vi "Stop Core.vi"(10 "final error code":i32, 11 "WebSocket Connection in":refnum<class "WebSocket Connection.lvclass">) -> (3 "WebSocket Connection out":refnum<class "WebSocket Connection.lvclass">)   [LabVIEW 2021, in "WebSocket Actors.lvlib" / "WebSocket Connection.lvclass"]
doc: "(<B>Filename</B>: Actor Framework.lvlib:Actor.lvclass:Stop Core.vi)\n\nDefines what the actor does before it stops. Use the <B>final error code</B> input to determine whether the actor shut down in response to an error.\n\nBy default, this method does nothing. A descendant class may override it to define behavior, such as shutting down any processes the actor initiated in its override of the Actor Core method."
uses:
  WebSocket Connection.lvclass
  Abstract Messages/WebSocket Connection Handler Msg/typedefs/Message Data.ctl
  <vilib>/ActorFramework/Message Enqueuer/Message Enqueuer.lvclass
  <vilib>/LS Instruments AG/LV-WebSockets/Data Format.ctl
  WebSocket Connection.lvclass/WebSocket Connection.ctl
  Abstract Messages/WebSocket Connection Handler Msg/properties/Connection Event.ctl
  <vilib>/LS Instruments AG/LV-WebSockets/StatusCode.ctl
  Abstract Messages/WebSocket Connection Handler Msg/WebSocket Connection Handler Msg.lvclass/WebSocket Connection Handler Msg.ctl
  <vilib>/ActorFramework/Message Enqueuer/Message Enqueuer.lvclass/Message Enqueuer.ctl
  <vilib>/ActorFramework/Message Enqueuer/Enqueue.vi
  Abstract Messages/WebSocket Connection Handler Msg/WebSocket Connection Handler Msg.lvclass
  C:/Program Files/National Instruments/LabVIEW 2021/vi.lib/ActorFramework/Message/Message.lvclass
  <vilib>/Utility/LVClass/Get LV Class Name.vi
  <resource>/AFDebug/Generate Trace for Message.vi
  <vilib>/ActorFramework/Message Priority Queue/Priority Enqueue.vi
  <vilib>/ActorFramework/Actor/Actor.lvclass
  <vilib>/LS Instruments AG/LV-WebSockets/LV WebSockets.lvlib
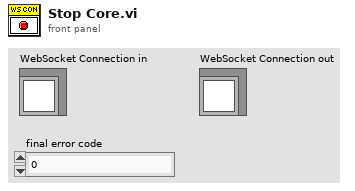
[diagram p1: front panel]
types:
  T1 = typedef "WebSocket Actors.lvlib/WebSocket Connection Handler Msg.lvclass/Message Data.ctl" = cluster{"Data":string, "Peer ID":string, "Connection Enqueuer":refnum<class "Message Enqueuer.lvclass">, "Data Format":T2}
  T2 = typedef "LV WebSockets.lvlib/Data Format.ctl" = enum16{"Text", "Binary"}
  T3 = typedef "WebSocket Actors.lvlib/WebSocket Connection.lvclass/Connection Status.ctl" = enum16{"Open", "Closed by Self", "Closed by Peer", "Dropped"}
  T4 = typedef "WebSocket Actors.lvlib/WebSocket Connection Handler Msg.lvclass/Connection Event.ctl" = enum16{"On Connect", "On Message", "On Close", "On Drop"}
  T5 = typedef "LV WebSockets.lvlib/StatusCode.ctl" = u16
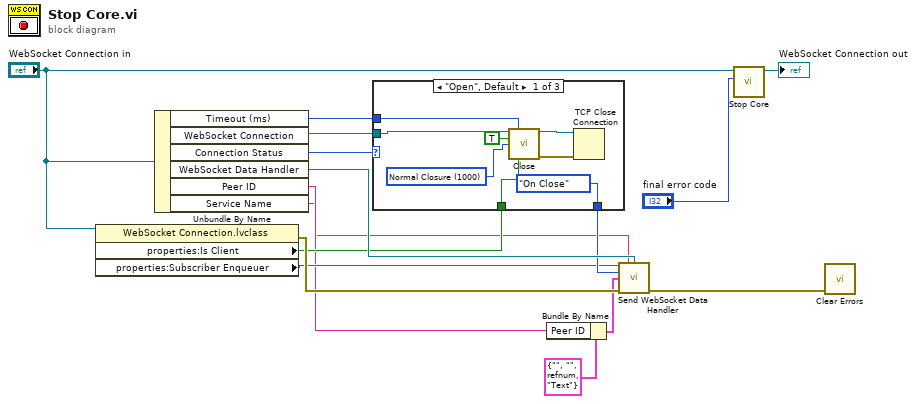
[diagram p0: block diagram]
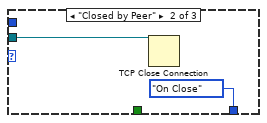
[diagram p2: hidden frame]
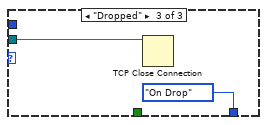
[diagram p3: hidden frame]
diagram:
  n1 = property class="WebSocket Connection.lvclass"(reference="WebSocket Connection in") -> (error out=w8:errorcluster, "properties:Is Client"=w6:bool, "properties:Subscriber Enqueuer"=w7:refnum<class "Message Enqueuer.lvclass">)  [unwired: 1 in, 1 out]
  n2 = Unbundle By Name("WebSocket Connection in") -> ("Timeout (ms)"=w2:i32, "WebSocket Connection"=w14:refnum<k5>, "Connection Status"=w13:T3, "WebSocket Data Handler"=w12:refnum<class "WebSocket Connection Handler Msg.lvclass">, "Peer ID"=w4:string, "Service Name"=w1:string)
  n3 = case shown="\"Open\", Default" w13 {
    tunnel: w14 -> [w24 w26 w28]
    tunnel: [Connection_Event."On Close" ("Connection Event") Connection_Event."On Close" ("Connection Event") Connection_Event."On Drop" ("Connection Event")] -> w10
    tunnel: w6 -> [w18 _ _]
    tunnel: w2 -> [w17 _ _]
    frame "Open", Default {
      w19 = T5 1000 items=["Normal Closure"=1000, "Going Away"=1001, "Protocol Error"=1002, "Wrong Data Type"=1003, "Reserved 1004"=1004, "Reserved 1005"=1005, "Reserved 1006"=1006, "Non Consistent Data Type"=1007, "Policy Violation"=1008, "Message Too Big"=1009, "Extensions Negotiation Error"=1010, "Unexpected Condition"=1011, "Reserved 1015"=1015] ("Status Code")
      n4 = call <vilib>:"Close.vi"("WebSocket Connection in"=w24, "timeout ms (5000)"=w17, "Send Reason (F)"=TRUE, "Status Code"=w19, "Mask payload?"=w18) -> ("WebSocket Connection in"=w22:refnum<k5>, "error out"=w23:errorcluster)  [unwired: 9 in]
      n5 = TCP Close Connection(connection ID=w22, error in (no error)=w23) -> ()  [unwired: 1 in, 2 out]
    }
    frame "Closed by Peer" {
      n6 = TCP Close Connection(connection ID=w26) -> ()  [unwired: 2 in, 2 out]
    }
    frame "Dropped" {
      n7 = TCP Close Connection(connection ID=w28) -> ()  [unwired: 2 in, 2 out]
    }
  }
  n8 = Bundle By Name(cluster=T1 {"Data"="", "Peer ID"="", "Connection Enqueuer"=refnum, "Data Format"=enum."Text"} ("Connection Message Data"), "Peer ID"=w4) -> (w3:T1)
  n9 = call "Send WebSocket Data Handler.vi"("Message Enqueuer"=w7, "Service Name"=w1, "Message Type"=w12, "Connection Event"=w10, "Connection Message Data"=w3, "error in (no error)"=w8) -> ("error out"=w11:errorcluster)  [unwired: 8 in, 1 out]
  n10 = call-parent "Stop Core.vi"("final error code"="final error code", "Actor in"="WebSocket Connection in") -> ("Actor out"=→"WebSocket Connection out":refnum<class "WebSocket Connection.lvclass">)  [unwired: 9 in]
  n11 = call <vilib>:"Clear Errors.vi"("error in (no error)"=w11) -> ()  [unwired: 5 in, 2 out]
